vi "Stimulus.Open.vi"(8 "error in (no error)":errorcluster, 11 "State Variables":T1={"NIVS.BaseLogPath"=path "", "NIVS.SystemDefinitionFile"=path "", "NIVS.Events"={"SequenceEvent"=refnum, "SystemChangeEvent"=refnum, "WorkspaceEvent"=refnum}, "NIVS.SequenceState"=enum."Idle", "NIVS.GatewayIPAddress"="", "NIVS.DataLogSpecRef"=refnum, "NIVS.DataLogManagerRef"=refnum, "NIVS.LogSessionGUID"="", "NIVS.WorkspaceManager"=refnum, "NIVS.Deployed"=FALSE, "NIVS.ProfileRef"=refnum, "NIVS.ProfileCallback"=refnum, "NIVS.SystemStateRefs"={"CustDatRef"=refnum, "EvtRef"=refnum, "Target State User Event"=refnum}, "UI.Abort"=refnum, "UI.Pause"=refnum, "UI.EnableLogging"=refnum, "UI.Start"=refnum, "UI.LogChannels"=refnum, "UI.StartIteration"=refnum, "UI.StartStep"=refnum, "UI.Sequence"=refnum, "UI.PreviewMode"=refnum, "UI.Graph"=refnum, "UI.BaseFileName"=refnum, "UI.Profiles"=refnum, "UI.CurrentStep"=refnum, "UI.CurrentIteration"=refnum, "UI.TotalIterations"=refnum, "Sequence.AbortChannel"="", "Sequence.StepInfoChannel"="", "Sequence.Iterations"=0, "Sequence.IterationInfoChannel"="", "Sequence.#ofColumns"=0, "Events.State"=refnum, "Events.Test Result"=refnum, "Events.Progress"=refnum, "INI.Settings"={"Build Location"=path "C:/Simple Sequence Editor/SequenceRepo", "LoggingLocation"=path ""}, "UI.Skip"=refnum, "Sequence.SkipChannel"="", "Restart.Path"=path "", "UI.Duration"=refnum, "Sequence.DurationChannel"=""}) -> (0 "error out":errorcluster, 3 "State Variables":T1={"NIVS.BaseLogPath"=path "", "NIVS.SystemDefinitionFile"=path "", "NIVS.Events"={"SequenceEvent"=refnum, "SystemChangeEvent"=refnum, "WorkspaceEvent"=refnum}, "NIVS.SequenceState"=enum."Idle", "NIVS.GatewayIPAddress"="", "NIVS.DataLogSpecRef"=refnum, "NIVS.DataLogManagerRef"=refnum, "NIVS.LogSessionGUID"="", "NIVS.WorkspaceManager"=refnum, "NIVS.Deployed"=FALSE, "NIVS.ProfileRef"=refnum, "NIVS.ProfileCallback"=refnum, "NIVS.SystemStateRefs"={"CustDatRef"=refnum, "EvtRef"=refnum, "Target State User Event"=refnum}, "UI.Abort"=refnum, "UI.Pause"=refnum, "UI.EnableLogging"=refnum, "UI.Start"=refnum, "UI.LogChannels"=refnum, "UI.StartIteration"=refnum, "UI.StartStep"=refnum, "UI.Sequence"=refnum, "UI.PreviewMode"=refnum, "UI.Graph"=refnum, "UI.BaseFileName"=refnum, "UI.Profiles"=refnum, "UI.CurrentStep"=refnum, "UI.CurrentIteration"=refnum, "UI.TotalIterations"=refnum, "Sequence.AbortChannel"="", "Sequence.StepInfoChannel"="", "Sequence.Iterations"=0, "Sequence.IterationInfoChannel"="", "Sequence.#ofColumns"=0, "Events.State"=refnum, "Events.Test Result"=refnum, "Events.Progress"=refnum, "INI.Settings"={"Build Location"=path "C:/Simple Sequence Editor/SequenceRepo", "LoggingLocation"=path ""}, "UI.Skip"=refnum, "Sequence.SkipChannel"="", "Restart.Path"=path "", "UI.Duration"=refnum, "Sequence.DurationChannel"=""})   [LabVIEW 2015, in "Simple Sequence Tools - Execution.lvlib"]
uses:
  Simple Sequence Tools - Execution.lvlib
  Types/Main.StateVariables.ctl
  Types/Execute.UserEventRefs.ctl
  <vilib>/NI Veristand/Execution/Workspace/SystemStateRegEventRef.ctl
  <vilib>/NI Veristand/Execution/Workspace/Target State Info.ctl
  <vilib>/NI Veristand/Execution/Workspace/Target State.ctl
  Types/Execution.SequenceState.ctl
  <vilib>/NI Veristand/Execution/DataLogging/DataLoggingSpecification Ref.ctl
  NationalInstruments.VeriStand.ClientAPI
  <vilib>/NI Veristand/Execution/DataLogging/IDataLogging Ref.ctl
  <vilib>/NI Veristand/Execution/Workspace/WorkspaceAPI.ctl
  NationalInstruments.VeriStand.RealTimeSequenceDefinitionApi
  <vilib>/NI Veristand/Execution/Workspace/SystemStateEventRef.ctl
  Shared/Types/INI.Settings.ctl
  NationalInstruments.VeriStand.DataTypes
  <vilib>/NI Veristand/Execution/DataLogging/File Conflict Operation.ctl
  Shared/SubVIs/Main.Constants.vi
  <vilib>/NI Veristand/Execution/DataLogging/New Data Logging Specification (TDMS).vi
  <vilib>/NI Veristand/Execution/DataLogging/Set Data Logging Rate (Target Rate).vi
  <vilib>/NI Veristand/Execution/DataLogging/Set Start Trigger (Start Immediately).vi
  Shared/Simple Sequence Tools - Shared.lvlib
  <vilib>/NI Veristand/Execution/DataLogging/NI_VS Data Logging API.lvlib
  <vilib>/NI Veristand/Execution/Workspace/NI_VS Workspace ExecutionAPI.lvlib
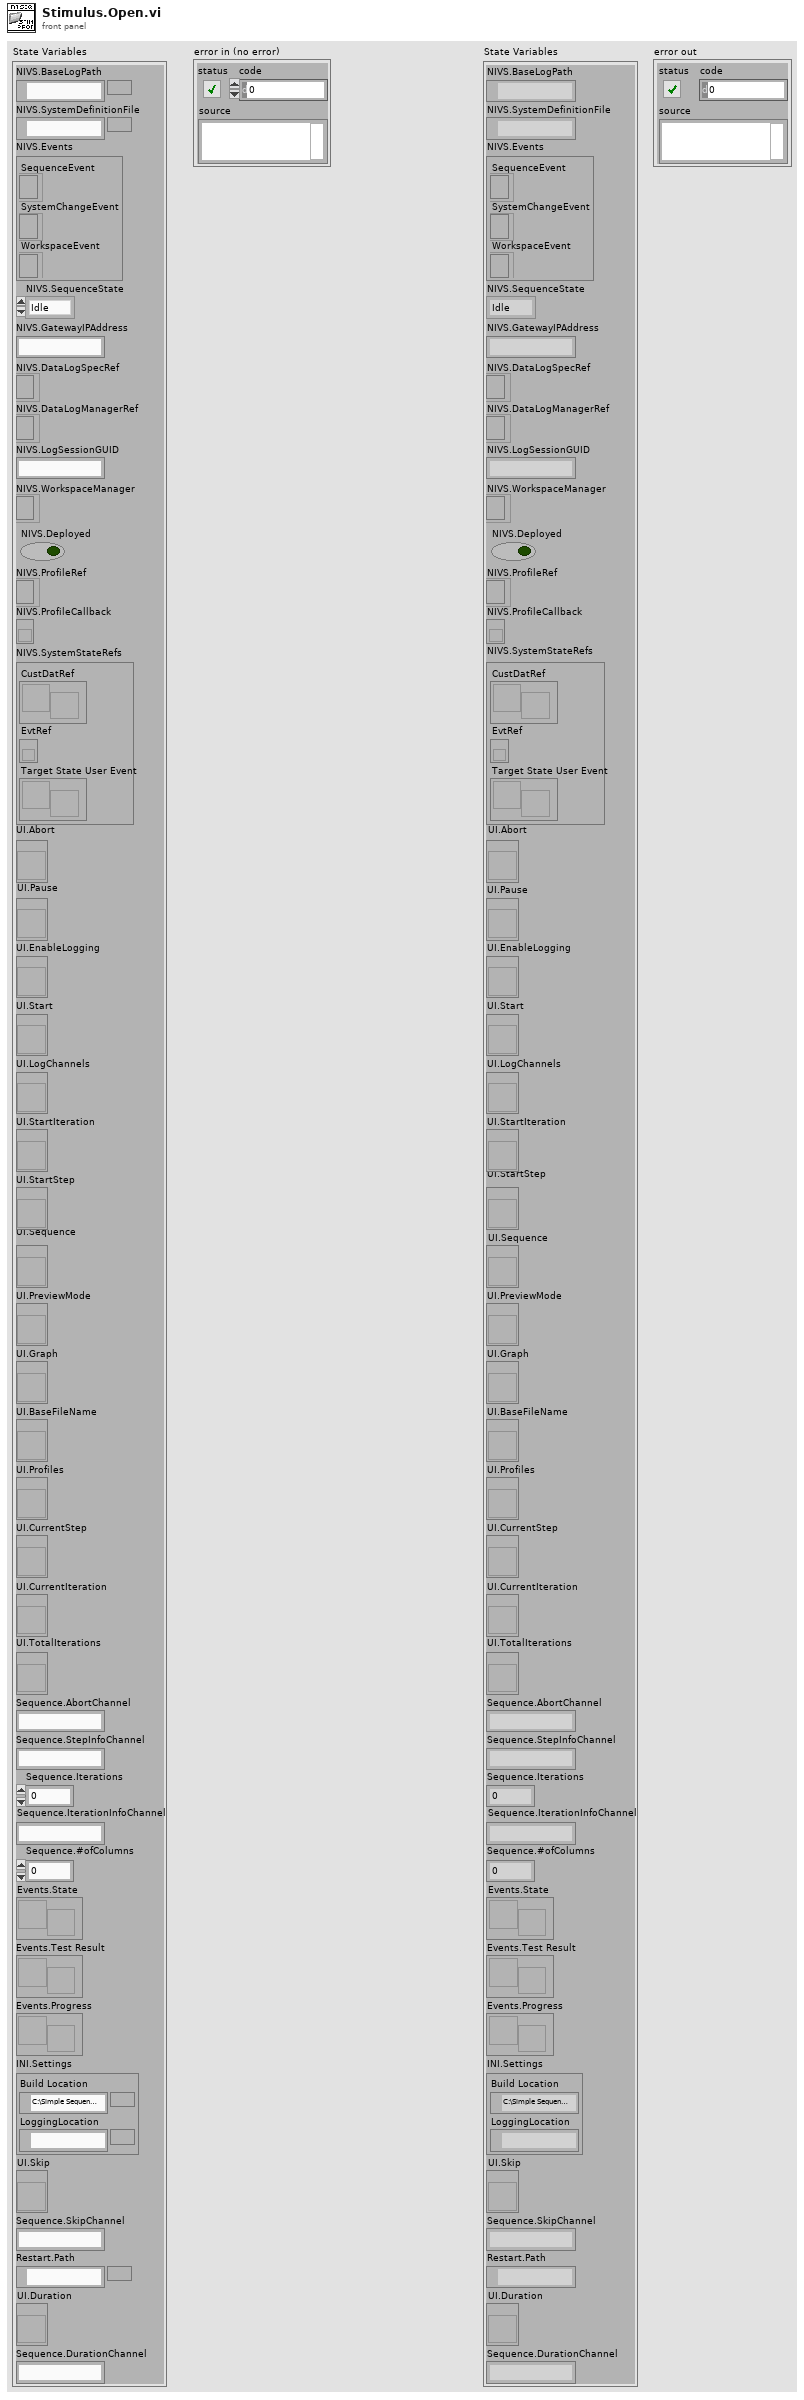
[diagram p1: front panel]
types:
  T1 = typedef "Simple Sequence Tools - Execution.lvlib/Main.StateVariables.ctl" = cluster{"NIVS.BaseLogPath":path, "NIVS.SystemDefinitionFile":path, "NIVS.Events":T2, "NIVS.SequenceState":T4, "NIVS.GatewayIPAddress":string, "NIVS.DataLogSpecRef":T5, "NIVS.DataLogManagerRef":T6, "NIVS.LogSessionGUID":string, "NIVS.WorkspaceManager":T7, "NIVS.Deployed":bool, "NIVS.ProfileRef":refnum<k24>, "NIVS.ProfileCallback":refnum<k27>, "NIVS.SystemStateRefs":T8, "UI.Abort":refnum<vi>, "UI.Pause":refnum<vi>, "UI.EnableLogging":refnum<vi>, "UI.Start":refnum<vi>, "UI.LogChannels":refnum<vi>, "UI.StartIteration":refnum<vi>, "UI.StartStep":refnum<vi>, "UI.Sequence":refnum<vi>, "UI.PreviewMode":refnum<vi>, "UI.Graph":refnum<vi>, "UI.BaseFileName":refnum<vi>, "UI.Profiles":refnum<vi>, "UI.CurrentStep":refnum<vi>, "UI.CurrentIteration":refnum<vi>, "UI.TotalIterations":refnum<vi>, "Sequence.AbortChannel":string, "Sequence.StepInfoChannel":string, "Sequence.Iterations":u32, "Sequence.IterationInfoChannel":string, "Sequence.#ofColumns":i32, "Events.State":refnum<user-event>, "Events.Test Result":refnum<user-event>, "Events.Progress":refnum<user-event>, "INI.Settings":T9, "UI.Skip":refnum<vi>, "Sequence.SkipChannel":string, "Restart.Path":path, "UI.Duration":refnum<vi>, "Sequence.DurationChannel":string}
  T2 = typedef "Simple Sequence Tools - Execution.lvlib/Execute.UserEventRefs.ctl" = cluster{"SequenceEvent":refnum<event-registration>, "SystemChangeEvent":T3, "WorkspaceEvent":refnum<event-registration>}
  T3 = typedef "NI_VS Workspace ExecutionAPI.lvlib/SystemStateRegEventRef.ctl" = refnum<event-registration>
  T4 = typedef "Simple Sequence Tools - Execution.lvlib/Execution.SequenceState.ctl" = enum16{"Idle", "Initializing", "Running", "Paused", "Finalizing", "Complete"}
  T5 = typedef "NI_VS Data Logging API.lvlib/DataLoggingSpecification Ref.ctl" = refnum<k24>
  T6 = typedef "NI_VS Data Logging API.lvlib/IDataLogging Ref.ctl" = refnum<k24>
  T7 = typedef "NI_VS Workspace ExecutionAPI.lvlib/WorkspaceAPI.ctl" = refnum<k24>
  T8 = typedef "NI_VS Workspace ExecutionAPI.lvlib/SystemStateEventRef.ctl" = cluster{"CustDatRef":refnum<user-event>, "EvtRef":refnum<k27>, "Target State User Event":refnum<user-event>}
  T9 = typedef "Simple Sequence Tools - Shared.lvlib/INI.Settings.ctl" = cluster{"Build Location":path, "LoggingLocation":path}
  T10 = typedef "Simple Sequence Tools - Execution.lvlib/Restart.Settings" = cluster{"LogFile":path, "Log Settings":T11[], "StimulusProfile":path, "StopIteration":u32, "StopStep":u32, "Log Channels":T15, "Base File Name":string, "Enable Logging":bool, "Profile":string, "StopDuration":dbl}
  T11 = typedef "NI_VS Data Logging API.lvlib/TDMS Channel Group.ctl" = cluster{"Group Name":string, "Group Description":string, "Group Properties":T12[], "Channels":T13[], "Time Channel Options":T14, "Time Channel Name":string}
  T12 = typedef "NI_VS Data Logging API.lvlib/TDMS Property.ctl" = cluster{"Name":string, "Value":variant}
  T13 = typedef "NI_VS Data Logging API.lvlib/TDMS Channel.ctl" = cluster{"Channel Name":string, "Channel Path":string, "Channel Description":string, "Channel Properties":T12[]}
  T14 = typedef "NI_VS Data Logging API.lvlib/Time Channel Options.ctl" = enum16{"No Time Channel", "Absolute Time", "System Time", "System Time - Microseconds", "Absolute Time as Double", "Relative To First Start Trigger", "Relative To Session Start"}
  T15 = typedef "Simple Sequence Tools - Execution.lvlib/Log.SelectedChannels.ctl" = enum16{"Channels (No System Channel)", "Aliases", "All"}
  T16 = typedef "NI_VS Data Logging API.lvlib/File Conflict Operation.ctl" = enum16{"Create Unique", "Append to Existing", "Overwrite"}
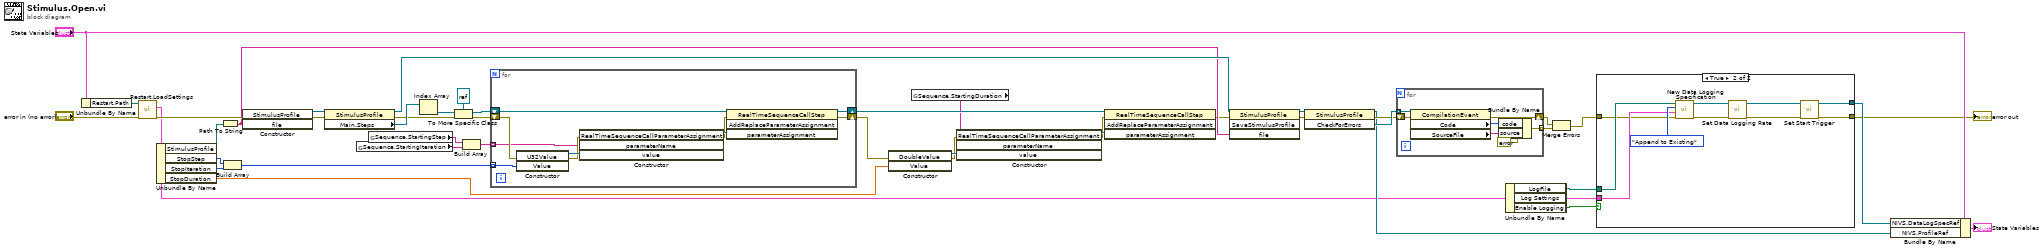
[diagram p0: block diagram]
diagram:
  n1 = Unbundle By Name("State Variables") -> ("Restart.Path"=w28:path)
  n2 = call "Restart.LoadSettings.vi"("error in"="error in (no error)", "path (use dialog)"=w28) -> ("error out"=w17:errorcluster, "Restart Settings"=w14:T10)  [unwired: 7 in, 1 out]
  n3 = Unbundle By Name(w14) -> ("StimulusProfile"=w25:path, "StopStep"=w26:u32, "StopIteration"=w27:u32, "StopDuration"=w2:dbl)
  n4 = Path To String(path=w25) -> (string=w15:string)
  n5 = Build Array(w26, w27) -> (w18:u32[])
  n6 = constructor class="StimulusProfile"(error in=w17, "file"=w15) -> (reference out=w43:refnum<k24>, error out=w42:errorcluster)  [unwired: 2 in, 2 out]
  n7 = property class="StimulusProfile"(reference=w43, error in=w42) -> (reference out=w33:refnum<k24>, error out=w21:errorcluster, "Main.Steps"=w24:refnum<k24>[])
  n8 = global read "Main.Constants.vi" "Sequence.StartingIteration"() -> (w34:string)
  n9 = global read "Main.Constants.vi" "Sequence.StartingStep"() -> (w35:string)
  n10 = Index Array(array=w24) -> (element=w23:refnum<k24>)  [unwired: 1 in]
  n11 = To More Specific Class(target class=refnum<k24> refnum ("new reference"), reference=w23, error in=w21) -> (specific class reference=w20:refnum<k24>, error out=w16:errorcluster)
  n12 = Build Array(w35, w34) -> (w19:string[])
  n13 = for {
    tunnel: w19 -> [w48] mode=indexing
    tunnel: w18 -> [w46] mode=indexing
    shift-right: [w53] -> w3
    shift-left: w20 -> [w54]
    shift-right: [w55] -> w4
    shift-left: w16 -> [w49]
    n14 = constructor class="U32Value"(error in=w49, "Value"=w46) -> (reference out=w51:refnum<k24>, error out=w50:errorcluster)  [unwired: 2 in, 2 out]
    n15 = constructor class="RealTimeSequenceCallParameterAs"(error in=w50, "parameterName"=w48, "value"=w51) -> (reference out=w52:refnum<k24>, error out=w47:errorcluster)  [unwired: 2 in, 3 out]
    n16 = invoke class="RealTimeSequenceCallStep" method="AddReplaceParameterAssignment"(reference=w54, error in=w47, "parameterAssignment"=w52) -> (reference out=w53:refnum<k24>, error out=w55:errorcluster)  [unwired: 1 in, 2 out]
  }
  n17 = constructor class="DoubleValue"(error in=w4, "Value"=w2) -> (reference out=w8:refnum<k24>, error out=w7:errorcluster)  [unwired: 2 in, 2 out]
  n18 = global read "Main.Constants.vi" "Sequence.StartingDuration"() -> (w1:string)
  n19 = constructor class="RealTimeSequenceCallParameterAs"(error in=w7, "parameterName"=w1, "value"=w8) -> (reference out=w9:refnum<k24>, error out=w6:errorcluster)  [unwired: 2 in, 3 out]
  n20 = invoke class="RealTimeSequenceCallStep" method="AddReplaceParameterAssignment"(reference=w3, error in=w6, "parameterAssignment"=w9) -> (error out=w5:errorcluster)  [unwired: 1 in, 3 out]
  n21 = invoke class="StimulusProfile" method="SaveStimulusProfile"(reference=w33, error in=w5, "file"=w15) -> (reference out=w41:refnum<k24>, error out=w40:errorcluster)  [unwired: 1 in, 2 out]
  n22 = invoke class="StimulusProfile" method="CheckForErrors"(reference=w41, error in=w40) -> (reference out=w31:refnum<k24>, error out=w38:errorcluster, "CheckForErrors"=w39:refnum<k24>[])  [unwired: 1 in]
  n23 = for {
    tunnel: w39 -> [w62] mode=indexing
    tunnel: [w57] -> w36 mode=indexing
    shift-right: [w56] -> w37
    shift-left: w38 -> [w61]
    n24 = property class="CompilationEvent"(reference=w62, error in=w61) -> (error out=w56:errorcluster, "Code"=w59:i32, "SourceFile"=w58:string)  [unwired: 1 out]
    n25 = Bundle By Name(cluster=errorcluster {"status"=TRUE, "code"=0, "source"=""} ("error out"), "code"=w59, "source"=w58) -> (w57:errorcluster)
  }
  n26 = Unbundle By Name(w14) -> ("LogFile"=w12:path, "Log Settings"=w10:T11[], "Enable Logging"=w13:bool)
  n27 = Merge Errors(w37, w36) -> (w11:errorcluster)
  n28 = case shown="True" w13 {
    tunnel: w11 -> [w63 w64]
    tunnel: [w63 w68] -> w30
    tunnel: [_ w67] -> w32
    tunnel: w12 -> [_ w66]
    tunnel: w10 -> [_ w65]
    frame False {
    }
    frame True {
      n29 = call-poly <vilib>:"New Data Logging Specification.vi"("error in (no error)"=w64, "Channel Groups"=w65, "File Conflict Operation"=File_Conflict_Operation."Append to Existing", "Base Log File Path"=w66) -> ("error out"=w70:errorcluster, "Data Logging Specification Ref out"=w73:T5)  [unwired: 6 in]
      n30 = call-poly <vilib>:"Set Data Logging Rate.vi"("error in (no error)"=w70, "Data Logging Specification Ref in"=w73) -> ("error out"=w71:errorcluster, "Data Logging Specification Ref out"=w72:T5)  [unwired: 8 in]
      n31 = call-poly <vilib>:"Set Start Trigger.vi"("error in (no error)"=w71, "Data Logging Specification Ref in"=w72) -> ("error out"=w68:errorcluster, "Data Logging Specification Ref out"=w67:T5)  [unwired: 8 in]
    }
  }
  "error out" <- w30
  n32 = Bundle By Name(cluster="State Variables", "NIVS.DataLogSpecRef"=w32, "NIVS.ProfileRef"=w31) -> (→"State Variables":T1)
